vi "Main.vi"(11 "Module Admin":refnum<class "Delacor_lib_QMH_Cloneable Module Admin.lvclass">) -> ()   [LabVIEW 2025, in "Sequencer.lvlib"]
doc: "This template is based off of the Queued Message Handler design pattern and the Queued Message Handler project template that ships with LabVIEW.\n\nThe main difference is that the queue is private to this module and communication between modules is performed via Broadcast and Request events.\n\nRequest events are wrapped in public API methods and are handled in the Event Handling Loop (EHL) of this VI. Any module can register for Broadcast events sent by this module. The EHL generates messages based on user interface actions.\n\nThe Message Handling Loop (MHL) processes messages generated by the EHL, or by other messages. The messages are string values, so new messages can be added easily to the Message Cases case structure in the MHL. Each message cluster can also provide an optional value for Message Data, which is a variant that can be converted to whatever message-specific data is required.\n_____\nBased on DQMH Dev Tools: Project Template 7.1.2.1547."
uses:
  Sequencer.lvlib
  <vilib>/Delacor/Delacor QMH/Libraries/Cloneable Module Admin_class/Delacor_lib_QMH_Cloneable Module Admin.lvclass
  C:/Program Files/National Instruments/LabVIEW 2025/vi.lib/Delacor/Delacor QMH/Libraries/Module Admin_class/Delacor_lib_QMH_Module Admin.lvclass
  Module Data--cluster.ctl
  <vilib>/Delacor/Delacor QMH/Libraries/Message Queue_class/Delacor_lib_QMH_Message Queue.lvclass/Delacor_lib_QMH_Message Queue.ctl
  <vilib>/Delacor/Delacor QMH/Libraries/Cloneable Module Admin_class/Delacor_lib_QMH_Cloneable Module Admin.lvclass/Delacor_lib_QMH_Cloneable Module Admin.ctl
  Stop Argument--cluster.ctl
  <vilib>/Delacor/Delacor QMH/Libraries/Module Admin_class/Delacor_lib_QMH_Module Admin.lvclass/Delacor_lib_QMH_Module Admin.ctl
  Get Modules Argument--cluster.ctl
  Get Modules (Reply Payload)--cluster.ctl
  Home Stepper Argument--cluster.ctl
  Home Stepper (Reply Payload)--cluster.ctl
  Go To Angle Argument--cluster.ctl
  Controls/Angle Indicator.ctl
  Controls/Motor Speed Slider.ctl
  Go To Angle (Reply Payload)--cluster.ctl
  Part Removal Position Argument--cluster.ctl
  Part Removal Position (Reply Payload)--cluster.ctl
  Torque Test Argument--cluster.ctl
  Controls/Sequencer/sequence array.ctl
  Controls/Sequencer/step cluster.ctl
  Torque Test (Reply Payload)--cluster.ctl
  Controls/Sequencer/results array.ctl
  Controls/Sequencer/results cluster.ctl
  <vilib>/Utility/miscctls.llb/LVPointTypeDef.ctl
  <vilib>/Delacor/Delacor QMH/Libraries/Message Queue_class/Delacor_lib_QMH_Enqueue Message (Single).vi
  <vilib>/Delacor/Delacor QMH/Libraries/Cloneable Module Admin_class/Delacor_lib_QMH_Get Module ID.vi
  <vilib>/Delacor/Delacor QMH/Libraries/Module Admin_class/Delacor_lib_QMH_Get External Launch.vi
  <vilib>/Analysis/baseanly.llb/Mean (DBL).vi
  <vilib>/Delacor/Delacor QMH/Libraries/Message Queue_class/Delacor_lib_QMH_Message Queue.lvclass
  USB IO/USB IO.lvlib
  Motor/Motor.lvlib
  <vilib>/Analysis/NI_AALBase.lvlib
  Wheatstone Bridge/Wheatstone Bridge.lvlib
panel:
  out "error out":errorcluster
  out "Status":string
  in  "Simulate EHL Error":bool
  in  "Simulate MHL Error":bool
  # "Other processes communicate with this Module via its Public API (wrappers for its Request Events).\n\nThis Module communicates with other processes via its Broadcast Events.\nAny process that wants to receive these messages can register for this module's Broadcast events."
  # "This template is for the DQMH framework. See the block diagram for more information on how to use this template."
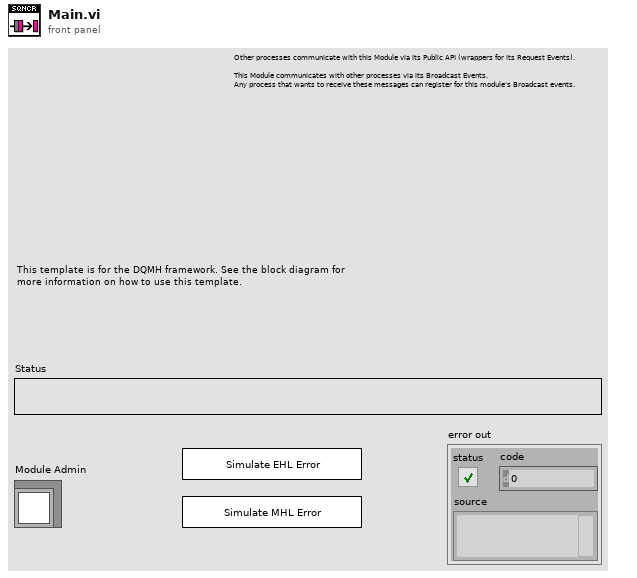
[diagram p1: front panel]
types:
  T1 = typedef "Sequencer.lvlib/Request Events--cluster.ctl" = cluster{"Stop Module":refnum<user-event>, "Show Panel":refnum<user-event>, "Hide Panel":refnum<user-event>, "Show Diagram":refnum<user-event>, "Get Module Execution Status":refnum<user-event>, "Get Modules":refnum<user-event>, "Home":refnum<user-event>, "Home Stepper":refnum<user-event>, "Go To Angle":refnum<user-event>, "Part Removal Position":refnum<user-event>, "Torque Test":refnum<user-event>}
  T2 = typedef "Sequencer.lvlib/Module Data--cluster.ctl" = cluster{"Status":string, "Modules":cluster{"Module IDs":i32[], "Module Names":string[]}}
  T3 = enum32{"invalid lock state", "Not Locked", "Locked (No Password)", "Password-protected"}
  T4 = typedef "Sequencer.lvlib/Stop Argument--cluster.ctl" = cluster{"Module ID":i32, "Origin":string, "Exit via Stop Module Req?":bool, "Wait for Module to stop?":bool}
  T5 = typedef "Sequencer.lvlib/Get Modules Argument--cluster.ctl" = cluster{"Module ID":i32, "Modules":cluster{"Module IDs":i32[], "Module Names":string[]}, "Wait Notifier":refnum<notifier>, "wait for reply":bool}
  T6 = typedef "Sequencer.lvlib/Home Stepper Argument--cluster.ctl" = cluster{"Module ID":i32, "Wait Notifier":refnum<notifier>, "wait for reply":bool}
  T7 = typedef "Sequencer.lvlib/Go To Angle Argument--cluster.ctl" = cluster{"Module ID":i32, "Angle":T8, "Speed [rpm]":T9, "Wait Notifier":refnum<notifier>, "wait for reply":bool}
  T8 = typedef "Angle Indicator.ctl" = dbl
  T9 = typedef "Motor Speed Slider.ctl" = dbl
  T10 = typedef "Sequencer.lvlib/Part Removal Position Argument--cluster.ctl" = cluster{"Module ID":i32, "Wait Notifier":refnum<notifier>, "wait for reply":bool}
  T11 = typedef "Sequencer.lvlib/Torque Test Argument--cluster.ctl" = cluster{"Module ID":i32, "Array 2":T12, "Speed [rpm]":T9, "On Time [ms]":dbl, "Wait Notifier":refnum<notifier>, "wait for reply":bool}
  T12 = typedef "sequence array.ctl" = T13[]
  T13 = typedef "step cluster.ctl" = cluster{"Angle Min [°]":dbl, "Angle Max [°]":dbl, "Torque Min [oz-in]":dbl, "Torque Max [oz-in]":dbl}
  T14 = typedef "LVPointTypeDef.ctl" = cluster{"Horizontal":i16, "Vertical":i16}
  T15 = enum32{"Invalid", "Standard", "Closed", "Hidden", "Minimized", "Maximized"}
  T16 = typedef "Sequencer.lvlib/Get Modules (Reply Payload)--cluster.ctl" = cluster{"Module ID":i32, "error":errorcluster}
  T17 = typedef "Sequencer.lvlib/Home Stepper (Reply Payload)--cluster.ctl" = cluster{"Module ID":i32, "Complete?":bool, "error":errorcluster}
  T18 = typedef "Sequencer.lvlib/Go To Angle (Reply Payload)--cluster.ctl" = cluster{"Module ID":i32, "Complete?":bool, "error":errorcluster}
  T19 = typedef "Sequencer.lvlib/Part Removal Position (Reply Payload)--cluster.ctl" = cluster{"Module ID":i32, "Completed?":bool, "error":errorcluster}
  T20 = typedef "Sequencer.lvlib/Torque Test (Reply Payload)--cluster.ctl" = cluster{"Module ID":i32, "Array 2":T21, "Complete?":bool, "error":errorcluster}
  T21 = typedef "results array.ctl" = T22[]
  T22 = typedef "results cluster.ctl" = cluster{"Angle [°]":dbl, "Torque [oz-in]":dbl, "Pass?":bool}
  T23 = cluster{"Module IDs":i32[], "Module Names":string[]}
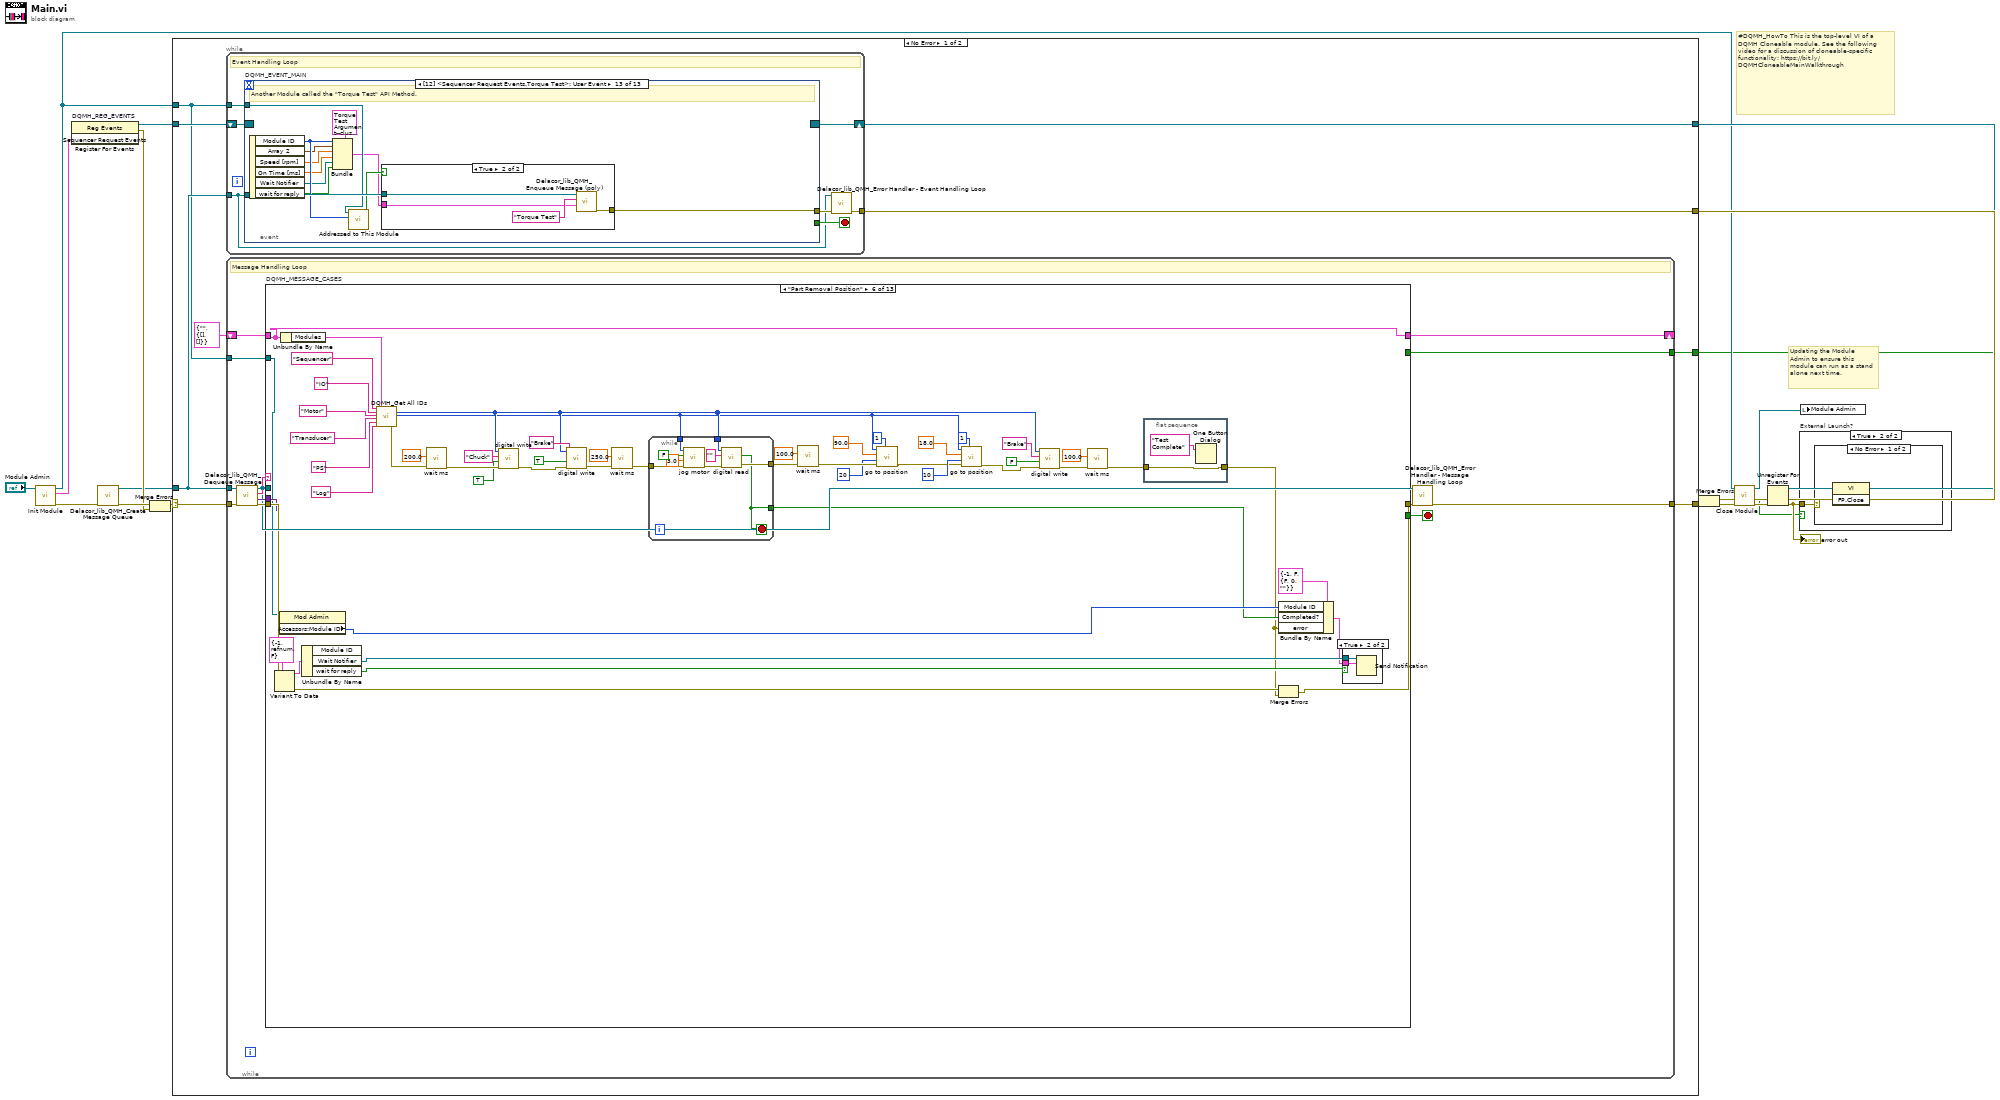
[diagram p0: block diagram]
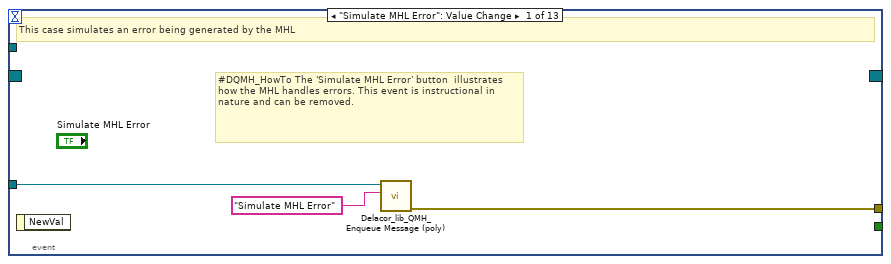
[diagram p2: hidden frame]
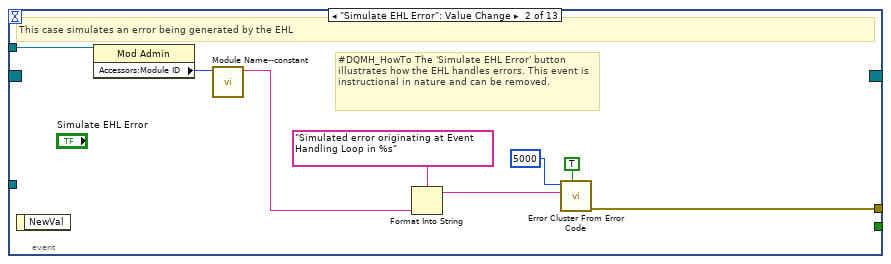
[diagram p3: hidden frame]
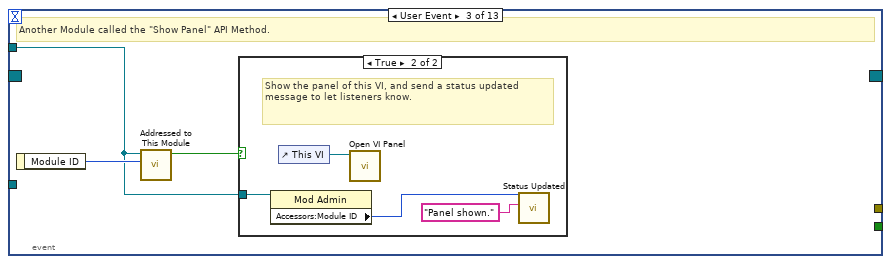
[diagram p4: hidden frame]
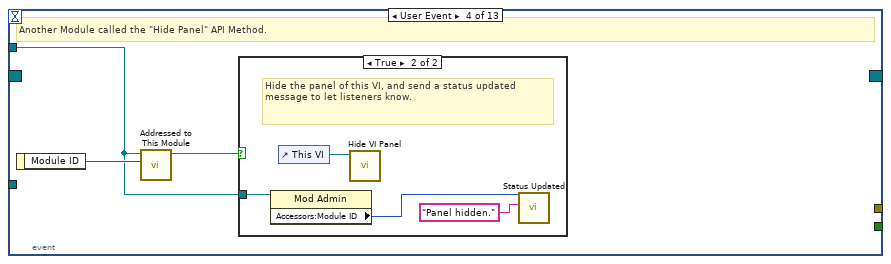
[diagram p6: hidden frame]
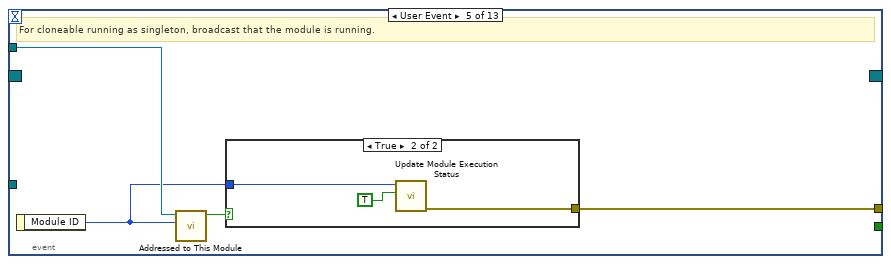
[diagram p8: hidden frame]
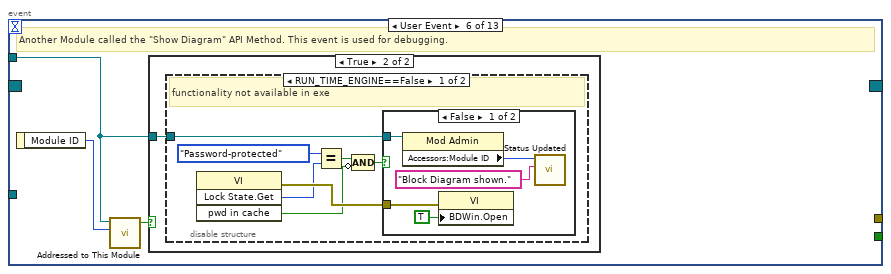
[diagram p10: hidden frame]
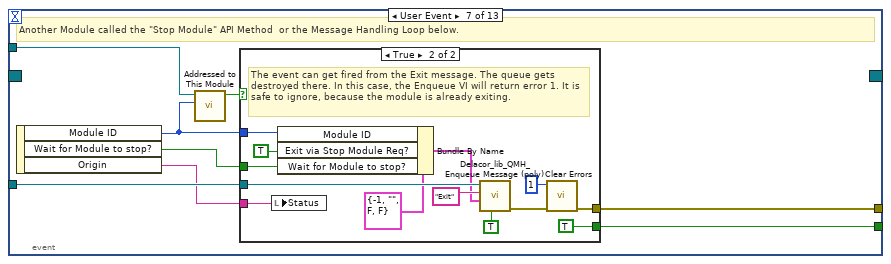
[diagram p14: hidden frame]
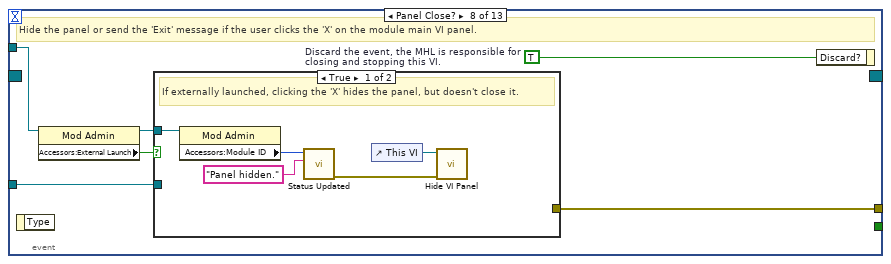
[diagram p16: hidden frame]
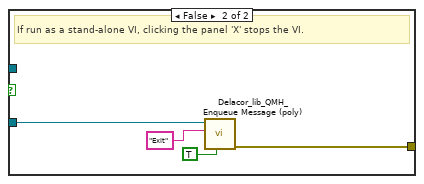
[diagram p17: hidden frame]
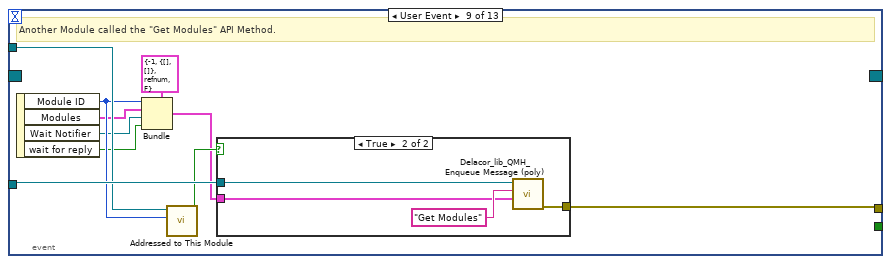
[diagram p18: hidden frame]
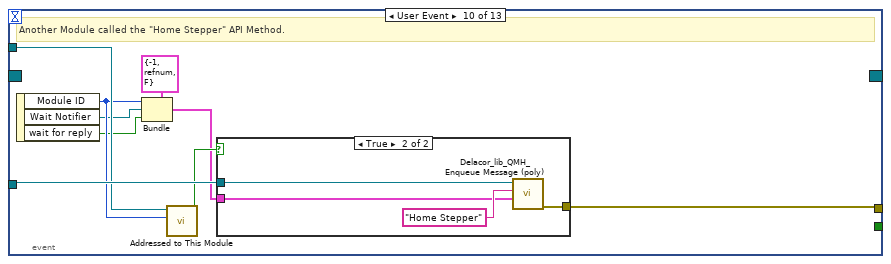
[diagram p20: hidden frame]
diagram:
  # "#DQMH_HowTo This is the top-level VI of a DQMH Cloneable module. See the following video for a discussion of cloneable-specific functionality: https://bit.ly/DQMHCloneableMainWalkthrough"
  # "Updating the Module Admin to ensure this module can run as a stand alone next time."
  n1 = call "Init Module.vi"("Cloneable Module Admin in"="Module Admin") -> ("error out"=w15:errorcluster, "Sequencer Request Events"=w7:T1, "Cloneable Module Admin out"=w4:refnum<class "Delacor_lib_QMH_Cloneable Module Admin.lvclass">)  [unwired: 8 in]
  n2 = register-events "DQMH_REG_EVENTS"(w7) -> (reference out=w8:refnum<event-registration>, error out=w10:errorcluster)  [unwired: 2 in]
  n3 = call <vilib>:"Delacor_lib_QMH_Create Message Queue.vi"("error in"=w15) -> ("error out"=w12:errorcluster, "Message Queue"=w6:refnum<class "Delacor_lib_QMH_Message Queue.lvclass">)  [unwired: 9 in]
  n4 = Merge Errors(w12, w10) -> (w11:errorcluster)
  n5 = case shown="No Error" w11 {
    selector: w11 -> [w25 w595]
    tunnel: [w27 w594] -> w16
    tunnel: [w24 w593] -> w9
    tunnel: w8 -> [w22 w593]
    tunnel: w6 -> [w21 w586]
    tunnel: [w26 _] -> w17
    tunnel: w4 -> [w20 w589]
    tunnel: [w19 _] -> w2
    frame No Error {
      n6 = while {
        tunnel: w21 -> [w28]
        shift-right: [w31] -> w24
        shift-left: w22 -> [w32]
        tunnel: [w33] -> w26
        tunnel: w20 -> [w29]
        stop <- w30 stop-if-true
        # "Event Handling Loop"
        n7 = event "DQMH_EVENT_MAIN" shown="[12] <Sequencer Request Events.Torque Test>: User Event" {
          selector: w32 -> [_ _ _ _ _ _ _ _ _ _ _ _ _]
          dyn-events: [_ _ _ _ _ _ _ _ _ _ _ _ _] -> w31
          timeout: _ -> [_ _ _ _ _ _ _ _ _ _ _ _ _]
          tunnel: [_ _ _ _ _ _ w86 _ _ _ _ _ _] -> w30
          tunnel: w28 -> [w36 _ _ _ _ _ w89 w106 w128 w141 w156 w169 w185]
          tunnel: [w37 w45 _ _ w63 _ w90 w109 w119 w133 w146 w161 w174] -> w34
          tunnel: w29 -> [_ w44 w46 w53 w61 w67 w88 w107 w126 w139 w154 w167 w183]
          event "Simulate MHL Error": Value Change {
            # "#DQMH_HowTo The 'Simulate MHL Error' button  illustrates how the MHL handles errors. This event is instructional in nature and can be removed."
            # "This case simulates an error being generated by the MHL"
            n8 = event-data() -> ()  [unwired: 1 in, 1 out]
            n9 = call-poly <vilib>:"Delacor_lib_QMH_Enqueue Message (poly).vi"("Message"="Simulate MHL Error", "Message Queue in"=w36) -> ("error out"=w37:errorcluster)  [unwired: 8 in, 1 out]
          }
          event "Simulate EHL Error": Value Change {
            # "#DQMH_HowTo The 'Simulate EHL Error' button  illustrates how the EHL handles errors. This event is instructional in nature and can be removed."
            # "This case simulates an error being generated by the EHL"
            n10 = event-data() -> ()  [unwired: 1 in, 1 out]
            n11 = property on="Property Node" class="Mod Admin"(reference=w44) -> ("Accessors:Module ID"=w43:i32)  [unwired: 1 in, 2 out]
            n12 = call "Module Name--constant.vi"("Module ID"=w43) -> ("Module Name"=w38:string)  [unwired: 10 in]
            n13 = Format Into String(format string="Simulated error originating at Event Handling Loop in %s", w38) -> (resulting string=w41:string)  [unwired: 2 in, 1 out]
            n14 = call <vilib>:"Error Cluster From Error Code.vi"("show call chain? (False)"=TRUE, "error message (\"\")"=w41, "error code (0)"=5000) -> ("error out"=w45:errorcluster)  [unwired: 6 in]
          }
          event User Event {
            # "Another Module called the \"Show Panel\" API Method."
            n15 = event-data() -> ("Module ID"=w47:i32)  [unwired: 1 in]
            n16 = call "Addressed to This Module.vi"("Module ID from Argument"=w47, "Module Admin"=w46) -> ("Addressed to this instance?"=w48:bool)  [unwired: 8 in, 1 out]
            n17 = case shown="True" w48 {
              tunnel: w46 -> [_ w50]
              frame False {
              }
              frame True {
                # "Show the panel of this VI, and send a status updated message to let listeners know."
                n18 = property on="Property Node" class="Mod Admin"(reference=w50) -> ("Accessors:Module ID"=w49:i32)  [unwired: 1 in, 2 out]
                n19 = control-ref of="This VI"() -> (w52:refnum<vi>)
                n20 = call "Open VI Panel.vi"("VI"=w52) -> ()  [unwired: 10 in, 1 out]
                n21 = call "Status Updated.vi"("Status"="Panel shown." ("format string"), "Module ID"=w49) -> ()  [unwired: 9 in, 1 out]
              }
            }
          }
          event User Event {
            # "Another Module called the \"Hide Panel\" API Method."
            n22 = event-data() -> ("Module ID"=w54:i32)  [unwired: 1 in]
            n23 = call "Addressed to This Module.vi"("Module ID from Argument"=w54, "Module Admin"=w53) -> ("Addressed to this instance?"=w55:bool)  [unwired: 8 in, 1 out]
            n24 = case shown="True" w55 {
              tunnel: w53 -> [_ w57]
              frame False {
              }
              frame True {
                # "Hide the panel of this VI, and send a status updated message to let listeners know."
                n25 = property on="Property Node" class="Mod Admin"(reference=w57) -> ("Accessors:Module ID"=w56:i32)  [unwired: 1 in, 2 out]
                n26 = control-ref of="This VI"() -> (w59:refnum<vi>)
                n27 = call "Hide VI Panel.vi"("VI"=w59) -> ()  [unwired: 10 in, 1 out]
                n28 = call "Status Updated.vi"("Status"="Panel hidden." ("format string"), "Module ID"=w56) -> ()  [unwired: 9 in, 1 out]
              }
            }
          }
          event User Event {
            # "For cloneable running as singleton, broadcast that the module is running."
            n29 = event-data() -> ("Module ID"=w60:i32)  [unwired: 1 in]
            n30 = call "Addressed to This Module.vi"("Module ID from Argument"=w60, "Module Admin"=w61) -> ("Addressed to this instance?"=w62:bool)  [unwired: 8 in, 1 out]
            n31 = case shown="True" w62 {
              tunnel: [_ w66] -> w63
              tunnel: w60 -> [_ w65]
              frame False {
              }
              frame True {
                n32 = call "Update Module Execution Status.vi"("Running?"=TRUE, "Module ID"=w65) -> ("error out"=w66:errorcluster)  [unwired: 9 in]
              }
            }
          }
          event User Event {
            # "Another Module called the \"Show Diagram\" API Method. This event is used for debugging."
            n33 = event-data() -> ("Module ID"=w68:i32)  [unwired: 1 in]
            n34 = call "Addressed to This Module.vi"("Module ID from Argument"=w68, "Module Admin"=w67) -> ("Addressed to this instance?"=w69:bool)  [unwired: 8 in, 1 out]
            n35 = case shown="True" w69 {
              tunnel: w67 -> [_ w70]
              frame False {
              }
              frame True {
                n36 = disable-structure shown="RUN_TIME_ENGINE==False" {
                  disable-tunnel: w70 -> [w71 _]
                  frame condition #0 (active) {
                    # "functionality not available in exe"
                    n37 = invoke on="Invoke Node" class="VI" method="Lock State.Get"() -> (error out=w77:errorcluster, "Get Lock State"=w76:T3, "pwd in cache"=w73:bool)  [unwired: 4 in, 1 out]
                    n38 = Equal?(x=T3."Password-protected", y=w76) -> (x = y?=w74:bool)
                    n39 = Compound Arithmetic op=AND(w74, invert w73) -> (w72:bool)
                    n40 = case shown="False" w72 {
                      tunnel: w77 -> [w82 _]
                      tunnel: w71 -> [w79 _]
                      frame False {
                        n41 = property on="Property Node" class="Mod Admin"(reference=w79) -> ("Accessors:Module ID"=w78:i32)  [unwired: 1 in, 2 out]
                        n42 = property on="Property Node" class="VI"(error in=w82, "BDWin.Open"=TRUE ("Block Diagram Window:Open")) -> ()  [unwired: 1 in, 2 out]
                        n43 = call "Status Updated.vi"("Status"="Block Diagram shown." ("format string"), "Module ID"=w78) -> ()  [unwired: 9 in, 1 out]
                      }
                      frame True {
                        # "Password-protected VI, and the password is not in the cache. Do not show the diagram."
                      }
                    }
                  }
                  frame condition #1 {
                  }
                }
              }
            }
          }
          event User Event {
            # "Another Module called the \"Stop Module\" API Method  or the Message Handling Loop below."
            n44 = event-data() -> ("Module ID"=w84:i32, "Wait for Module to stop?"=w85:bool, "Origin"=w83:string)  [unwired: 1 in]
            n45 = call "Addressed to This Module.vi"("Module ID from Argument"=w84, "Module Admin"=w88) -> ("Addressed to this instance?"=w87:bool)  [unwired: 8 in, 1 out]
            n46 = case shown="True" w87 {
              tunnel: [_ w102] -> w90
              tunnel: w89 -> [_ w98]
              tunnel: [_ TRUE] -> w86
              tunnel: w85 -> [_ w93]
              tunnel: w84 -> [_ w95]
              tunnel: w83 -> [_ w91]
              frame False {
              }
              frame True {
                # "The event can get fired from the Exit message. The queue gets destroyed there. In this case, the Enqueue VI will return error 1. It is safe to ignore, because the module is already exiting."
                n47 = local write "Status"(w91) -> ()
                n48 = Bundle By Name(cluster=T4 {"Module ID"=-1, "Origin"="", "Exit via Stop Module Req?"=FALSE, "Wait for Module to stop?"=FALSE} ("Stop Argument"), "Module ID"=w95, "Exit via Stop Module Req?"=TRUE, "Wait for Module to stop?"=w93) -> (w92:T4)
                n49 = call-poly <vilib>:"Delacor_lib_QMH_Enqueue Message (poly).vi"("Priority Message? (F)"=TRUE, "Message Data"=w92, "Message"="Exit", "Message Queue in"=w98) -> ("error out"=w103:errorcluster)  [unwired: 6 in, 1 out]
                n50 = call <vilib>:"Clear Errors.vi"("error in (no error)"=w103, "specific error code to clear (0: all)"=1) -> ("error out"=w102:errorcluster)  [unwired: 4 in, 1 out]
              }
            }
          }
          event Panel Close? {
            w108 = TRUE  # Discard the event, the MHL is responsible for closing and stopping this VI.
            # "Hide the panel or send the 'Exit' message if the user clicks the 'X' on the module main VI panel."
            n51 = event-data() -> ()  [unwired: 1 in, 1 out]
            n52 = property on="Property Node" class="Mod Admin"(reference=w107) -> (reference out=w104:refnum<class "Delacor_lib_QMH_Cloneable Module Admin.lvclass">, "Accessors:External Launch"=w105:bool)  [unwired: 1 in, 1 out]
            n53 = case shown="True" w105 {
              tunnel: w106 -> [_ w117]
              tunnel: [_ w118] -> w109
              tunnel: w104 -> [w112 _]
              frame True {
                # "If externally launched, clicking the 'X' hides the panel, but doesn't close it."
                n54 = property on="Property Node" class="Mod Admin"(reference=w112) -> ("Accessors:Module ID"=w111:i32)  [unwired: 1 in, 2 out]
                n55 = call "Status Updated.vi"("Status"="Panel hidden." ("format string"), "Module ID"=w111) -> ("error out"=w110:errorcluster)  [unwired: 9 in]
                n56 = control-ref of="This VI"() -> (w114:refnum<vi>)
                n57 = call "Hide VI Panel.vi"("error in"=w110, "VI"=w114) -> ()  [unwired: 9 in, 1 out]
              }
              frame False {
                # "If run as a stand-alone VI, clicking the panel 'X' stops the VI."
                n58 = call-poly <vilib>:"Delacor_lib_QMH_Enqueue Message (poly).vi"("Priority Message? (F)"=TRUE, "Message"="Exit", "Message Queue in"=w117) -> ("error out"=w118:errorcluster)  [unwired: 7 in, 1 out]
              }
            }
            n59 = event-data ("Event Filter Node")("Discard?"=w108) -> ()  [unwired: 1 in, 1 out]
          }
          event User Event {
            # "Another Module called the \"Get Modules\" API Method."
            n60 = event-data() -> ("Module ID"=w123:i32, "Modules"=w122:T23, "Wait Notifier"=w121:refnum<notifier>, "wait for reply"=w120:bool)  [unwired: 1 in]
            n61 = Bundle(cluster=T5 {"Module ID"=-1, "Modules"={"Module IDs"=[], "Module Names"=[]}, "Wait Notifier"=refnum, "wait for reply"=FALSE} ("Get Modules Argument"), "Module ID"=w123, "Modules"=w122, "Wait Notifier"=w121, "wait for reply"=w120) -> (w124:T5)
            n62 = call "Addressed to This Module.vi"("Module ID from Argument"=w123, "Module Admin"=w126) -> ("Addressed to this instance?"=w127:bool)  [unwired: 8 in, 1 out]
            n63 = case shown="True" w127 {
              tunnel: w128 -> [_ w132]
              tunnel: w124 -> [_ w130]
              tunnel: [_ w129] -> w119
              frame False {
              }
              frame True {
                n64 = call-poly <vilib>:"Delacor_lib_QMH_Enqueue Message (poly).vi"("Message Data"=w130, "Message"="Get Modules", "Message Queue in"=w132) -> ("error out"=w129:errorcluster)  [unwired: 7 in, 1 out]
              }
            }
          }
          event User Event {
            # "Another Module called the \"Home Stepper\" API Method."
            n65 = event-data() -> ("Module ID"=w136:i32, "Wait Notifier"=w135:refnum<notifier>, "wait for reply"=w134:bool)  [unwired: 1 in]
            n66 = Bundle(cluster=T6 {"Module ID"=-1, "Wait Notifier"=refnum, "wait for reply"=FALSE} ("Home Stepper Argument"), "Module ID"=w136, "Wait Notifier"=w135, "wait for reply"=w134) -> (w137:T6)
            n67 = call "Addressed to This Module.vi"("Module ID from Argument"=w136, "Module Admin"=w139) -> ("Addressed to this instance?"=w140:bool)  [unwired: 8 in, 1 out]
            n68 = case shown="True" w140 {
              tunnel: w141 -> [_ w145]
              tunnel: w137 -> [_ w143]
              tunnel: [_ w142] -> w133
              frame False {
              }
              frame True {
                n69 = call-poly <vilib>:"Delacor_lib_QMH_Enqueue Message (poly).vi"("Message Data"=w143, "Message"="Home Stepper", "Message Queue in"=w145) -> ("error out"=w142:errorcluster)  [unwired: 7 in, 1 out]
              }
            }
          }
          event User Event {
            # "Another Module called the \"Go To Angle\" API Method."
            n70 = event-data() -> ("Module ID"=w151:i32, "Angle"=w150:T8, "Speed [rpm]"=w149:T9, "Wait Notifier"=w148:refnum<notifier>, "wait for reply"=w147:bool)  [unwired: 1 in]
            n71 = Bundle(cluster=T7 {"Module ID"=-1, "Angle"=0.0, "Speed [rpm]"=9.818181818181818, "Wait Notifier"=refnum, "wait for reply"=FALSE} ("Go To Angle Argument"), "Module ID"=w151, "Angle"=w150, "Speed [rpm]"=w149, "Wait Notifier"=w148, "wait for reply"=w147) -> (w152:T7)
            n72 = call "Addressed to This Module.vi"("Module ID from Argument"=w151, "Module Admin"=w154) -> ("Addressed to this instance?"=w155:bool)  [unwired: 8 in, 1 out]
            n73 = case shown="True" w155 {
              tunnel: w156 -> [_ w160]
              tunnel: w152 -> [_ w158]
              tunnel: [_ w157] -> w146
              frame False {
              }
              frame True {
                n74 = call-poly <vilib>:"Delacor_lib_QMH_Enqueue Message (poly).vi"("Message Data"=w158, "Message"="Go To Angle", "Message Queue in"=w160) -> ("error out"=w157:errorcluster)  [unwired: 7 in, 1 out]
              }
            }
          }
          event User Event {
            # "Another Module called the \"Part Removal Position\" API Method."
            n75 = event-data() -> ("Module ID"=w164:i32, "Wait Notifier"=w163:refnum<notifier>, "wait for reply"=w162:bool)  [unwired: 1 in]
            n76 = Bundle(cluster=T10 {"Module ID"=-1, "Wait Notifier"=refnum, "wait for reply"=FALSE} ("Part Removal Position Argument"), "Module ID"=w164, "Wait Notifier"=w163, "wait for reply"=w162) -> (w165:T10)
            n77 = call "Addressed to This Module.vi"("Module ID from Argument"=w164, "Module Admin"=w167) -> ("Addressed to this instance?"=w168:bool)  [unwired: 8 in, 1 out]
            n78 = case shown="True" w168 {
              tunnel: w169 -> [_ w173]
              tunnel: w165 -> [_ w171]
              tunnel: [_ w170] -> w161
              frame False {
              }
              frame True {
                n79 = call-poly <vilib>:"Delacor_lib_QMH_Enqueue Message (poly).vi"("Message Data"=w171, "Message"="Part Removal Position", "Message Queue in"=w173) -> ("error out"=w170:errorcluster)  [unwired: 7 in, 1 out]
              }
            }
          }
          event User Event {
            # "Another Module called the \"Torque Test\" API Method."
            n80 = event-data() -> ("Module ID"=w180:i32, "Array 2"=w179:T12, "Speed [rpm]"=w178:T9, "On Time [ms]"=w177:dbl, "Wait Notifier"=w176:refnum<notifier>, "wait for reply"=w175:bool)  [unwired: 1 in]
            n81 = Bundle(cluster=T11 {"Module ID"=-1, "Array 2"=[], "Speed [rpm]"=9.818181818181818, "On Time [ms]"=0.0, "Wait Notifier"=refnum, "wait for reply"=FALSE} ("Torque Test Argument"), "Module ID"=w180, "Array 2"=w179, "Speed [rpm]"=w178, "On Time [ms]"=w177, "Wait Notifier"=w176, "wait for reply"=w175) -> (w181:T11)
            n82 = call "Addressed to This Module.vi"("Module ID from Argument"=w180, "Module Admin"=w183) -> ("Addressed to this instance?"=w184:bool)  [unwired: 8 in, 1 out]
            n83 = case shown="True" w184 {
              tunnel: w185 -> [_ w189]
              tunnel: w181 -> [_ w187]
              tunnel: [_ w186] -> w174
              frame False {
              }
              frame True {
                n84 = call-poly <vilib>:"Delacor_lib_QMH_Enqueue Message (poly).vi"("Message Data"=w187, "Message"="Torque Test", "Message Queue in"=w189) -> ("error out"=w186:errorcluster)  [unwired: 7 in, 1 out]
              }
            }
          }
        }
        n85 = call-dynamic "Delacor_lib_QMH_Error Handler - Event Handling Loop.vi"("error in"=w34, "Message Queue in"=w28) -> ("dup error in"=w33:errorcluster)  [unwired: 8 in, 1 out]
      }
      n86 = while {
        tunnel: w21 -> [w190]
        shift-right: [w197] -> _
        shift-left: T2 {"Status"="", "Modules"={"Module IDs"=[], "Module Names"=[]}} ("Data Cluster") -> [w198]
        tunnel: w25 -> [w201]
        tunnel: [w199] -> w27
        tunnel: w20 -> [w192]
        tunnel: [w191] -> w19
        stop <- w196 stop-if-true
        # "Message Handling Loop"
        n87 = call-dynamic "Delacor_lib_QMH_Dequeue Message.vi"("error in"=w201, "Message Queue in"=w190) -> ("error out"=w200:errorcluster, "Message Data"=w194:variant, "Message"=w195:string, "Message Queue out"=w193:refnum<class "Delacor_lib_QMH_Message Queue.lvclass">)  [unwired: 6 in]
        n88 = case "DQMH_MESSAGE_CASES" shown="\"Part Removal Position\"" w195 {
          selector: w195 -> [_ _ _ _ _ _ _ _ _ _ _ _ w575]
          tunnel: w193 -> [_ _ _ _ _ _ _ _ _ w530 _ w567 _]
          tunnel: w200 -> [w221 w225 w241 w299 w328 w410 w464 w525 w527 w539 w556 w573 w584]
          tunnel: [w219 w225 w232 w290 w319 w401 w455 w524 w527 w535 w555 w568 w585] -> w202
          tunnel: w198 -> [w212 w224 w229 w261 w316 w391 w434 w523 w526 w534 w553 w566 w582]
          tunnel: [w211 w224 w228 w261 w311 w391 w434 w523 w526 w534 w553 w566 w582] -> w197
          tunnel: [_ _ _ _ _ _ _ _ _ _ _ w565 _] -> w196
          tunnel: w194 -> [_ _ w239 w297 w326 w408 w462 _ _ w533 _ w563 _]
          tunnel: w192 -> [w207 _ w230 w288 w317 w399 w453 _ _ w532 w551 w558 w581]
          tunnel: [_ _ _ _ _ _ _ _ _ _ _ w561 _] -> w191
          frame "Initialize" {
            w204 = "Initial Message" ("Initial Message")
            # "#DQMH_CodeNeeded - Initialize the appearance of the front panel."
            # "#DQMH_CodeNeeded - Initialize your state data here."
            # "Initialize - Any operation that needs to be done before the module can receive messages. Synchronize Caller Events.vi will inform Start Module.vi that the module has launched and is ready to receive messages. Module Did Init.vi will broadcast that the module initialized."
            n89 = call "Synchronize Caller Events.vi"("error in"=w221, "Module Admin"=w207) -> ("error out"=w220:errorcluster, "Module Admin out"=w206:refnum<class "Delacor_lib_QMH_Cloneable Module Admin.lvclass">)  [unwired: 8 in]
            n90 = property on="Property Node" class="Mod Admin"(reference=w206) -> ("Accessors:Module ID"=w203:i32, "Accessors:External Launch"=w208:bool)  [unwired: 1 in, 2 out]
            n91 = call "Module Name--constant.vi"("Module ID"=w203) -> ("Module Name"=w216:string)  [unwired: 10 in]
            n92 = property on="Property Node" class="VI"("Front Panel.Title"=w216) -> (reference out=w218:refnum<vi>, error out=w223:errorcluster)  [unwired: 2 in]
            n93 = Select(t=T15."Hidden" ("State"), s=w208, f=T15."Standard" ("State")) -> (s? t:f=w213:T15)
            n94 = invoke on="Invoke Node" class="VI" method="FP.Open"(reference=w218, error in=w223, "State"=w213) -> (reference out=w217:refnum<vi>, error out=w222:errorcluster)  [unwired: 2 in, 3 out]
            n95 = Bundle By Name(cluster=w212, "Status"=w204) -> (w211:T2)
            n96 = invoke on="Invoke Node" class="VI" method="FP.Center"(reference=w217, error in=w222) -> ()  [unwired: 1 in, 3 out]
            n97 = property on="Pane" class="Pane"("Origin"=T14 {"Horizontal"=0, "Vertical"=0}) -> ()  [unwired: 2 in, 2 out]
            n98 = call "Module Name--constant.vi"("Module ID"=w203) -> ("Module Name"=w209:string)  [unwired: 10 in]
            n99 = call "Module Did Init.vi"("error in"=w220, "Initialized?"=TRUE, "Origin"=w209, "Module ID"=w203) -> ("error out"=w219:errorcluster)  [unwired: 7 in]
            "Status" <- w204
          }
          frame "---Module Specific---" {
            # "Separator -- The following cases handle messages specific to this Module."
          }
          frame "Get Modules" {
            n100 = property class="Mod Admin"(reference=w230) -> ("Accessors:Module ID"=w231:i32)  [unwired: 1 in, 2 out]
            n101 = Variant To Data(error in=w241, type=T5 {"Module ID"=-1, "Modules"={"Module IDs"=[], "Module Names"=[]}, "Wait Notifier"=refnum, "wait for reply"=FALSE} ("Get Modules Argument"), Variant=w239) -> (data=w237:T5, error out=w240:errorcluster)
            n102 = Unbundle By Name(w237) -> ("Modules"=w227:T23, "Wait Notifier"=w236:refnum<notifier>, "wait for reply"=w235:bool)  [unwired: 1 out]
            n103 = in-place {
              in-place-border: w227 -> [w243]
              in-place-border: [errorcluster {"status"=FALSE, "code"=0, "source"=""} ("error")] -> w226
              n104 = in-place-cluster #1(w229) -> ()  [unwired: 1 out]
              n105 = in-place-cluster #1("Modules"=w243) -> (w228:T2)
            }
            n106 = Bundle By Name(cluster=T16 {"Module ID"=-1, "error"={"status"=FALSE, "code"=0, "source"=""}} ("Get Modules (Reply Payload)"), "Module ID"=w231, "error"=w226) -> (w234:T16)
            n107 = Merge Errors(w240, w226) -> (w232:errorcluster)
            n108 = case "DQMH_FIRE_NOTIFIER" shown="True" w235 {
              tunnel: w236 -> [_ w245]
              tunnel: w234 -> [_ w244]
              frame False {
              }
              frame True {
                n109 = Send Notification(notification=w244, notifier=w245) -> ()  [unwired: 1 in, 2 out]
              }
            }
          }
          frame "Home Stepper" {
            w251 = 10 ("Pause Time [ms]")
            n110 = property class="Mod Admin"(reference=w288) -> ("Accessors:Module ID"=w289:i32)  [unwired: 1 in, 2 out]
            n111 = Variant To Data(error in=w299, type=T6 {"Module ID"=-1, "Wait Notifier"=refnum, "wait for reply"=FALSE} ("Home Stepper Argument"), Variant=w297) -> (data=w295:T6, error out=w298:errorcluster)
            n112 = Unbundle By Name(w261) -> ("Modules"=w287:T23)
            n113 = Unbundle By Name(w295) -> ("Wait Notifier"=w294:refnum<notifier>, "wait for reply"=w293:bool)  [unwired: 1 out]
            n114 = call "DQMH_Get All IDs.vi"("Module 1"="Sequencer" ("Module Name"), "Module 2"="IO" ("Module Name"), "Module 3"="Motor" ("Module Name"), "Module 4"="Transducer" ("Module Name"), "Module 5"="PS" ("Module Name"), "Module 6"="Log" ("Module Name"), "Modules"=w287) -> ("error out"=w280:errorcluster, "Module 2"=w260:i32, "Module 3"=w246:i32)  [unwired: 6 in, 4 out]
            n115 = call "wait ms.vi"("error in"=w280, "ms (1000)"=200.0) -> ("error out"=w274:errorcluster)  [unwired: 9 in]
            n116 = call "digital write.vi"("error in"=w274, "On/Off"=TRUE, "Line"="Chuck", "Module ID"=w260) -> ("error out"=w273:errorcluster)  [unwired: 6 in, 1 out]
            n117 = call "digital write.vi"("error in"=w273, "On/Off"=TRUE, "Line"="Brake", "Module ID"=w260) -> ("error out"=w276:errorcluster)  [unwired: 6 in, 1 out]
            n118 = call "wait ms.vi"("error in"=w276, "ms (1000)"=250.0) -> ("error out"=w275:errorcluster)  [unwired: 9 in]
            n119 = while {
              tunnel: w275 -> [w308]
              tunnel: w246 -> [w305]
              tunnel: w260 -> [w303]
              tunnel: [w301] -> w248
              tunnel: [w300] -> w249
              stop <- w300 stop-if-true
              n120 = call "jog motor.vi"("error in"=w308, "Speed [rpm]"=2.0, "CCW? (T)"=FALSE, "Module ID"=w305) -> ("error out"=w304:errorcluster)  [unwired: 5 in, 2 out]
              n121 = call "digital read.vi"("error in"=w304, "Line"="", "Module ID"=w303) -> ("error out"=w301:errorcluster, "High/Low"=w300:bool)  [unwired: 6 in, 1 out]
            }
            n122 = call "zero.vi"("error in"=w248, "Module ID"=w246) -> ("error out"=w247:errorcluster)  [unwired: 8 in, 1 out]
            n123 = call "go to position.vi"("Pause Time [ms]"=w251, "error in"=w247, "Velocity [rpm]"=10, "Position"=100.0, "Module ID"=w246) -> ("error out"=w254:errorcluster)  [unwired: 4 in, 2 out]
            n124 = call "go to position.vi"("Pause Time [ms]"=w251, "error in"=w254, "Velocity [rpm]"=5, "Position"=10.0, "Module ID"=w246) -> ("error out"=w250:errorcluster)  [unwired: 4 in, 2 out]
            n125 = call "wait ms.vi"("error in"=w250, "ms (1000)"=100.0) -> ("error out"=w267:errorcluster)  [unwired: 9 in]
            n126 = call "digital write.vi"("error in"=w267, "On/Off"=FALSE, "Line"="Chuck", "Module ID"=w260) -> ("error out"=w265:errorcluster)  [unwired: 6 in, 1 out]
            n127 = call "digital write.vi"("error in"=w265, "On/Off"=FALSE, "Line"="Brake", "Module ID"=w260) -> ("error out"=w262:errorcluster)  [unwired: 6 in, 1 out]
            n128 = call "wait ms.vi"("error in"=w262, "ms (1000)"=100.0) -> ("error out"=w259:errorcluster)  [unwired: 9 in]
            n129 = call "zero.vi"("error in"=w259, "Module ID"=w246) -> ("error out"=w258:errorcluster)  [unwired: 8 in, 1 out]
            n130 = Bundle By Name(cluster=T17 {"Module ID"=-1, "Complete?"=FALSE, "error"={"status"=FALSE, "code"=0, "source"=""}} ("Home Stepper (Reply Payload)"), "Module ID"=w289, "Complete?"=w249, "error"=w258) -> (w292:T17)
            n131 = Merge Errors(w298, w258) -> (w290:errorcluster)
            n132 = case "DQMH_FIRE_NOTIFIER" shown="True" w293 {
              tunnel: w294 -> [_ w310]
              tunnel: w292 -> [_ w309]
              frame False {
              }
              frame True {
                n133 = Send Notification(notification=w309, notifier=w310) -> ()  [unwired: 1 in, 2 out]
              }
            }
          }
          frame "Go To Angle" {
            n134 = Variant To Data(error in=w328, type=T7 {"Module ID"=-1, "Angle"=0.0, "Speed [rpm]"=9.818181818181818, "Wait Notifier"=refnum, "wait for reply"=FALSE} ("Go To Angle Argument"), Variant=w326) -> (data=w324:T7, error out=w327:errorcluster)
            n135 = property class="Mod Admin"(reference=w317) -> ("Accessors:Module ID"=w318:i32)  [unwired: 1 in, 2 out]
            n136 = Unbundle By Name(w324) -> ("Angle"=w315:T8, "Speed [rpm]"=w314:T9, "Wait Notifier"=w323:refnum<notifier>, "wait for reply"=w322:bool)  [unwired: 1 out]
            n137 = in-place {
              in-place-border: w315 -> [w340]
              in-place-border: w314 -> [w339]
              in-place-border: [w331] -> w312
              n138 = in-place-cluster #2(w316) -> ("Modules"=w330:T23)
              n139 = call "DQMH_Get All IDs.vi"("Module 1"="Sequencer" ("Module Name"), "Module 2"="IO" ("Module Name"), "Module 3"="Motor" ("Module Name"), "Module 4"="Transducer" ("Module Name"), "Module 5"="PS" ("Module Name"), "Module 6"="Log" ("Module Name"), "Modules"=w330) -> ("error out"=w351:errorcluster, "Module 2"=w334:i32, "Module 3"=w341:i32)  [unwired: 6 in, 4 out]
              n140 = call "wait ms.vi"("error in"=w351, "ms (1000)"=250.0) -> ("error out"=w350:errorcluster)  [unwired: 9 in]
              n141 = call "digital write.vi"("error in"=w350, "On/Off"=TRUE, "Line"="Brake", "Module ID"=w334) -> ("error out"=w347:errorcluster)  [unwired: 6 in, 1 out]
              n142 = call "digital write.vi"("error in"=w347, "On/Off"=FALSE, "Line"="Chuck", "Module ID"=w334) -> ("error out"=w344:errorcluster)  [unwired: 6 in, 1 out]
              n143 = call "wait ms.vi"("error in"=w344, "ms (1000)"=250.0) -> ("error out"=w342:errorcluster)  [unwired: 9 in]
              n144 = call "go to position.vi"("Pause Time [ms]"=10, "error in"=w342, "Velocity [rpm]"=w339, "Position"=w340, "Module ID"=w341) -> ("error out"=w337:errorcluster)  [unwired: 4 in, 2 out]
              n145 = call "digital write.vi"("error in"=w337, "On/Off"=FALSE, "Line"="Brake", "Module ID"=w334) -> ("error out"=w333:errorcluster)  [unwired: 6 in, 1 out]
              n146 = call "wait ms.vi"("error in"=w333, "ms (1000)"=50.0) -> ("error out"=w331:errorcluster)  [unwired: 9 in]
              n147 = in-place-cluster #2("Modules"=w330) -> (w311:T2)
            }
            n148 = Not(x=w312) -> (.not. x?=w313:bool)
            n149 = Bundle By Name(cluster=T18 {"Module ID"=-1, "Complete?"=FALSE, "error"={"status"=FALSE, "code"=0, "source"=""}} ("Go To Angle (Reply Payload)"), "Module ID"=w318, "Complete?"=w313, "error"=w312) -> (w321:T18)
            n150 = Merge Errors(w327, w312) -> (w319:errorcluster)
            n151 = case "DQMH_FIRE_NOTIFIER" shown="True" w322 {
              tunnel: w323 -> [_ w359]
              tunnel: w321 -> [_ w358]
              frame False {
              }
              frame True {
                n152 = Send Notification(notification=w358, notifier=w359) -> ()  [unwired: 1 in, 2 out]
              }
            }
          }
          frame "Part Removal Position" {
            n153 = Variant To Data(error in=w410, type=T10 {"Module ID"=-1, "Wait Notifier"=refnum, "wait for reply"=FALSE} ("Part Removal Position Argument"), Variant=w408) -> (data=w406:T10, error out=w409:errorcluster)
            n154 = property class="Mod Admin"(reference=w399) -> ("Accessors:Module ID"=w400:i32)  [unwired: 1 in, 2 out]
            n155 = Unbundle By Name(w391) -> ("Modules"=w392:T23)
            n156 = Unbundle By Name(w406) -> ("Wait Notifier"=w405:refnum<notifier>, "wait for reply"=w404:bool)  [unwired: 1 out]
            n157 = call "DQMH_Get All IDs.vi"("Module 1"="Sequencer" ("Module Name"), "Module 2"="IO" ("Module Name"), "Module 3"="Motor" ("Module Name"), "Module 4"="Transducer" ("Module Name"), "Module 5"="PS" ("Module Name"), "Module 6"="Log" ("Module Name"), "Modules"=w392) -> ("error out"=w373:errorcluster, "Module 2"=w374:i32, "Module 3"=w362:i32)  [unwired: 6 in, 4 out]
            n158 = call "wait ms.vi"("error in"=w373, "ms (1000)"=200.0) -> ("error out"=w385:errorcluster)  [unwired: 9 in]
            n159 = call "digital write.vi"("error in"=w385, "On/Off"=TRUE, "Line"="Chuck", "Module ID"=w374) -> ("error out"=w384:errorcluster)  [unwired: 6 in, 1 out]
            n160 = call "digital write.vi"("error in"=w384, "On/Off"=TRUE, "Line"="Brake", "Module ID"=w374) -> ("error out"=w387:errorcluster)  [unwired: 6 in, 1 out]
            n161 = call "wait ms.vi"("error in"=w387, "ms (1000)"=250.0) -> ("error out"=w386:errorcluster)  [unwired: 9 in]
            n162 = while {
              tunnel: w386 -> [w421]
              tunnel: w362 -> [w418]
              tunnel: w374 -> [w416]
              tunnel: [w414] -> w381
              tunnel: [w413] -> w372
              stop <- w413 stop-if-true
              n163 = call "jog motor.vi"("error in"=w421, "Speed [rpm]"=3.0, "CCW? (T)"=FALSE, "Module ID"=w418) -> ("error out"=w417:errorcluster)  [unwired: 5 in, 2 out]
              n164 = call "digital read.vi"("error in"=w417, "Line"="", "Module ID"=w416) -> ("error out"=w414:errorcluster, "High/Low"=w413:bool)  [unwired: 6 in, 1 out]
            }
            n165 = call "wait ms.vi"("error in"=w381, "ms (1000)"=100.0) -> ("error out"=w371:errorcluster)  [unwired: 9 in]
            n166 = call "go to position.vi"("Pause Time [ms]"=1, "error in"=w371, "Velocity [rpm]"=20, "Position"=90.0, "Module ID"=w362) -> ("error out"=w365:errorcluster)  [unwired: 4 in, 2 out]
            n167 = call "go to position.vi"("Pause Time [ms]"=1, "error in"=w365, "Velocity [rpm]"=10, "Position"=18.0, "Module ID"=w362) -> ("error out"=w364:errorcluster)  [unwired: 4 in, 2 out]
            n168 = call "digital write.vi"("error in"=w364, "On/Off"=FALSE, "Line"="Brake", "Module ID"=w374) -> ("error out"=w376:errorcluster)  [unwired: 6 in, 1 out]
            n169 = call "wait ms.vi"("error in"=w376, "ms (1000)"=100.0) -> ("error out"=w361:errorcluster)  [unwired: 9 in]
            n170 = flat-sequence {
              tunnel: w361 -> [w411]
              tunnel: [w411] -> w360
              frame #0 {
                n171 = One Button Dialog(message="Test Complete") -> ()  [unwired: 1 in, 1 out]
              }
            }
            n172 = Bundle By Name(cluster=T19 {"Module ID"=-1, "Completed?"=FALSE, "error"={"status"=FALSE, "code"=0, "source"=""}} ("Part Removal Position (Reply Payload)"), "Module ID"=w400, "Completed?"=w372, "error"=w360) -> (w403:T19)
            n173 = Merge Errors(w409, w360) -> (w401:errorcluster)
            n174 = case "DQMH_FIRE_NOTIFIER" shown="True" w404 {
              tunnel: w405 -> [_ w423]
              tunnel: w403 -> [_ w422]
              frame False {
              }
              frame True {
                n175 = Send Notification(notification=w422, notifier=w423) -> ()  [unwired: 1 in, 2 out]
              }
            }
          }
          frame "Torque Test" {
            n176 = Variant To Data(error in=w464, type=T11 {"Module ID"=-1, "Array 2"=[], "Speed [rpm]"=9.818181818181818, "On Time [ms]"=0.0, "Wait Notifier"=refnum, "wait for reply"=FALSE} ("Torque Test Argument"), Variant=w462) -> (data=w460:T11, error out=w463:errorcluster)
            n177 = property class="Mod Admin"(reference=w453) -> ("Accessors:Module ID"=w454:i32)  [unwired: 1 in, 2 out]
            n178 = Unbundle By Name(w434) -> ("Modules"=w444:T23)
            n179 = Unbundle By Name(w460) -> ("Array 2"=w435:T12, "Speed [rpm]"=w432:T9, "On Time [ms]"=w430:dbl, "Wait Notifier"=w459:refnum<notifier>, "wait for reply"=w458:bool)  [unwired: 1 out]
            n180 = call "DQMH_Get All IDs.vi"("Module 1"="Sequencer" ("Module Name"), "Module 2"="IO" ("Module Name"), "Module 3"="Motor" ("Module Name"), "Module 4"="Transducer" ("Module Name"), "Module 5"="PS" ("Module Name"), "Module 6"="Log" ("Module Name"), "Modules"=w444) -> ("error out"=w445:errorcluster, "Module 2"=w431:i32, "Module 3"=w433:i32, "Module 4"=w424:i32)  [unwired: 6 in, 3 out]
            n181 = call "wait ms.vi"("error in"=w445, "ms (1000)"=200.0) -> ("error out"=w439:errorcluster)  [unwired: 9 in]
            n182 = call "digital write.vi"("error in"=w439, "On/Off"=TRUE, "Line"="Brake", "Module ID"=w431) -> ("error out"=w438:errorcluster)  [unwired: 6 in, 1 out]
            n183 = call "digital write.vi"("error in"=w438, "On/Off"=FALSE, "Line"="Chuck", "Module ID"=w431) -> ("error out"=w436:errorcluster)  [unwired: 6 in, 1 out]
            n184 = call "wait ms.vi"("error in"=w436, "ms (1000)"=250.0) -> ("error out"=w426:errorcluster)  [unwired: 9 in]
            n185 = disable-structure shown="Disabled" {
              disable-tunnel: w426 -> [w467 w468]
              disable-tunnel: [w466 w468] -> w425
              disable-tunnel: w424 -> [w465 _]
              frame Disabled {
                n186 = call "zero.vi"("error in"=w467, "Module ID"=w465) -> ("error out"=w466:errorcluster)  [unwired: 8 in, 1 out]
              }
              frame Enabled {
              }
            }
            n187 = for {
              tunnel: w435 -> [w505] mode=indexing
              tunnel: w433 -> [w488]
              tunnel: w432 -> [w499]
              tunnel: w431 -> [w484]
              tunnel: w424 -> [w492]
              tunnel: [w490] -> w429 mode=indexing
              tunnel: w430 -> [w470]
              shift-right: [w481] -> w428
              shift-left: w425 -> [w501]
              # "For Each Angle"
              n188 = Unbundle By Name(w505) -> ("Angle Min [°]"=w504:dbl, "Angle Max [°]"=w503:dbl, "Torque Min [oz-in]"=w478:dbl, "Torque Max [oz-in]"=w480:dbl)
              n189 = Build Array(w504, w503) -> (w502:dbl[])
              n190 = call-poly <vilib>:"Mean.vi"("X"=w502) -> ("mean"=w500:dbl)  [unwired: 1 out]
              n191 = call "go to position.vi"("Pause Time [ms]"=50, "error in"=w501, "Velocity [rpm]"=w499, "Position"=w500, "Module ID"=w488) -> ("error out"=w497:errorcluster)  [unwired: 4 in, 2 out]
              n192 = call "wait ms.vi"("error in"=w497, "ms (1000)"=20.0) -> ("error out"=w489:errorcluster)  [unwired: 9 in]
              n193 = call "read position.vi"("error in"=w489, "Module ID"=w488) -> ("error out"=w471:errorcluster, "Position"=w487:dbl)  [unwired: 7 in, 1 out]
              n194 = flat-sequence {
                tunnel: w471 -> [_]
                tunnel: w470 -> [w508]
                tunnel: [w509] -> w469
                frame #0 {
                  n195 = Get Date/Time In Seconds() -> (seconds since 1Jan1904=w510:timestamp)
                  n196 = Divide(x=w508, y=1000.0) -> (x/y=w506:dbl)
                  n197 = Add(x=w510, y=w506) -> (x+y=w509:timestamp)
                }
              }
              n198 = Initialize Array(0.0 ("element"), 1 ("dimension size")) -> (w475:dbl[])
              n199 = call "digital write.vi"("error in"=w471, "On/Off"=TRUE, "Line"="PS", "Module ID"=w484) -> ("error out"=w493:errorcluster)  [unwired: 6 in, 1 out]
              n200 = while {
                tunnel: w492 -> [w520]
                shift-right: [w518] -> w474
                shift-left: w475 -> [w519]
                tunnel: w471 -> [w515]
                tunnel: [w514] -> w472
                tunnel: w469 -> [w513]
                i -> [w517]
                stop <- w511 continue-if-true
                # "Torque Recording Loop"
                n201 = Get Date/Time In Seconds() -> (seconds since 1Jan1904=w512:timestamp)
                n202 = call "read dvr.vi"("error in"=w515, "Module ID"=w520) -> ("error out"=w514:errorcluster, "Numeric"=w516:dbl)  [unwired: 7 in, 1 out]
                n203 = Greater?(x=w513, y=w512) -> (0:w511:bool)
                n204 = Insert Into Array(array=w519, index=w517, new element=w516) -> (w518:dbl[])
              }
              n205 = call "wait ms.vi"("error in"=w493, "ms (1000)"=w470) -> ()  [unwired: 9 in, 1 out]
              n206 = call "wait ms.vi"("error in"=w472, "ms (1000)"=40.0) -> ("error out"=w485:errorcluster)  [unwired: 9 in]
              n207 = Array Max & Min(array=w474) -> (max value=w473:dbl)  [unwired: 3 out]
              n208 = call "digital write.vi"("error in"=w485, "On/Off"=FALSE, "Line"="PS", "Module ID"=w484) -> ("error out"=w481:errorcluster)  [unwired: 6 in, 1 out]
              n209 = In Range and Coerce(upper limit=w480, x=w473, lower limit=w478) -> (In Range?=w479:bool)  [unwired: 1 out]
              n210 = Bundle By Name(cluster=T22 {"Angle [°]"=0.0, "Torque [oz-in]"=0.0, "Pass?"=FALSE} ("Cluster"), "Angle [°]"=w487, "Torque [oz-in]"=w473, "Pass?"=w479) -> (w490:T22)
            }
            n211 = Bundle By Name(cluster=T20 {"Module ID"=-1, "Array 2"=[], "Complete?"=FALSE, "error"={"status"=FALSE, "code"=0, "source"=""}} ("Torque Test (Reply Payload)"), "Module ID"=w454, "Array 2"=w429, "Complete?"=TRUE, "error"=w428) -> (w457:T20)
            n212 = Merge Errors(w463, w428) -> (w455:errorcluster)
            n213 = case "DQMH_FIRE_NOTIFIER" shown="True" w458 {
              tunnel: w459 -> [_ w522]
              tunnel: w457 -> [_ w521]
              frame False {
              }
              frame True {
                n214 = Send Notification(notification=w521, notifier=w522) -> ()  [unwired: 1 in, 2 out]
              }
            }
          }
          frame "---Copy This Frame---" {
            # "Duplicate this frame when creating new messages.  Change this comment in the duplicated frame to describe this message."
            n215 = Merge Errors(w525) -> (w524:errorcluster)
          }
          frame "---Exit and Error Handling---" {
            # "Separator - the following cases handle errors and exit messages."
          }
          frame "Error" {
            # "#DQMH_CodeRecommended - If the module is running in standalone mode (External Launch = FALSE), this code will pop up an error dialog and call the 'Exit' message if an error occurs. Add more fine-grained error management here."
            # "Error - Check the error message data and respond accordingly. This message is sent by the \"Error Handler\" VIs at the end of each loop in this application."
            n216 = property on="Property Node" class="Mod Admin"(reference=w532) -> ("Accessors:External Launch"=w531:bool, "Accessors:Module ID"=w529:i32)  [unwired: 1 in, 2 out]
            n217 = Variant To Data(error in=w539, type=errorcluster {"status"=FALSE, "code"=0, "source"=""} ("error constant"), Variant=w533) -> (data=w528:errorcluster, error out=w537:errorcluster)
            n218 = local write "error out"(w528) -> ()
            n219 = call "Error Reported.vi"("Error"=w528, "Module ID"=w529) -> ()  [unwired: 9 in, 1 out]
            n220 = case shown="False" w531 {
              tunnel: [w544 _] -> w536
              tunnel: w530 -> [w542 _]
              tunnel: w528 -> [w543 _]
              frame False {
                n221 = disable-structure shown="Default" {
                  disable-tunnel: w543 -> [w545 _]
                  frame condition #0 (active) {
                    # "If the module is running standalone, then pop up an error dialog and call the \"Exit\" message."
                    n222 = call <vilib>:"Simple Error Handler.vi"("error in (no error)"=w545) -> ()  [unwired: 4 in, 5 out]
                  }
                  frame condition #1 {
                    # "To prevent the Simple Error Handler VI from being loaded (e.g. when deploying to a Real-Time target), add the Conditional Disable Symbol \"DQMH_Disable_SEH\" to your project and set it to TRUE."
                  }
                }
                n223 = call-poly <vilib>:"Delacor_lib_QMH_Enqueue Message (poly).vi"("Priority Message? (F)"=TRUE, "Message"="Exit", "Message Queue in"=w542) -> ("error out"=w544:errorcluster)  [unwired: 7 in, 1 out]
              }
              frame True {
                # "If the module was launched externally, calling the Error Reported broadcast VI is the only action performed by the \"Error\" message. The module's caller can then process the error appropriately."
              }
            }
            n224 = Merge Errors(w537, w536) -> (w535:errorcluster)
          }
          frame "Simulate MHL Error" {
            # "#DQMH_HowTo The 'Simulate MHL Error' button  illustrates how the MHL handles errors. This event is instructional in nature and can be removed."
            # "Simulate an error occurring at the MHL"
            n225 = property on="Property Node" class="Mod Admin"(reference=w551) -> ("Accessors:Module ID"=w552:i32)  [unwired: 1 in, 2 out]
            n226 = call "Module Name--constant.vi"("Module ID"=w552) -> ("Module Name"=w547:string)  [unwired: 10 in]
            n227 = Format Into String(format string="Simulated error originating at Message Handling Loop in %s", w547) -> (resulting string=w548:string)  [unwired: 2 in, 1 out]
            n228 = call <vilib>:"Error Cluster From Error Code.vi"("show call chain? (False)"=TRUE, "error message (\"\")"=w548, "error code (0)"=5001) -> ("error out"=w554:errorcluster)  [unwired: 6 in]
            n229 = Merge Errors(w556, w554) -> (w555:errorcluster)
          }
          frame "Exit" {
            w564 = 91  # 91: not all Exit messages will have an argument
            w565 = TRUE  # Stop the VI
            # "Release the message queue reference"
            # "#DQMH_CodeNeeded - Add any required cleanup code here."
            # "Exit - Exit the application."
            n230 = Variant To Data(error in=w573, type=T4 {"Module ID"=-1, "Origin"="", "Exit via Stop Module Req?"=FALSE, "Wait for Module to stop?"=FALSE} ("Stop Argument"), Variant=w563) -> (data=w560:T4, error out=w569:errorcluster)
            n231 = call <vilib>:"Clear Errors.vi"("error in (no error)"=w569, "specific error code to clear (0: all)"=w564) -> ("error out"=w572:errorcluster)  [unwired: 4 in, 1 out]
            n232 = property on="Property Node" class="Mod Admin"(reference=w558) -> ("Accessors:Module ID"=w557:i32)  [unwired: 1 in, 2 out]
            n233 = control-ref of="This VI"() -> (w559:refnum<vi>)
            n234 = call-dynamic "Delacor_lib_QMH_Release Message Queue.vi"("error in"=w572, "Message Queue"=w567) -> ("error out"=w571:errorcluster)  [unwired: 9 in]
            n235 = call "Handle Exit.vi"("Stop Argument"=w560, "Module Admin in"=w558, "VI reference"=w559) -> ("error out"=w570:errorcluster, "Wait for Stop?"=w561:bool)  [unwired: 7 in]
            n236 = Merge Errors(w571, w570) -> (w568:errorcluster)
            n237 = call "Error Reported.vi"("Error"=w568, "Module ID"=w557) -> ()  [unwired: 9 in, 1 out]
          }
          frame Default {
            # "'Default' case only runs if there is a message that isn't defined in any of the other cases.  Output a programming error."
            n238 = property on="Property Node" class="Mod Admin"(reference=w581) -> ("Accessors:Module ID"=w580:i32)  [unwired: 1 in, 2 out]
            n239 = call "Module Name--constant.vi"("Module ID"=w580) -> ("Module Name"=w574:string)  [unwired: 10 in]
            n240 = Format Into String(format string="The invalid message string \"%s\" was received in the Message Handling Loop for module \"%s\".", w575, w574) -> (resulting string=w577:string)  [unwired: 2 in, 1 out]
            n241 = call <vilib>:"Error Cluster From Error Code.vi"("show call chain? (False)"=TRUE, "error message (\"\")"=w577, "error code (0)"=1) -> ("error out"=w583:errorcluster)  [unwired: 6 in]
            n242 = Merge Errors(w584, w583) -> (w585:errorcluster)
          }
        }
        n243 = call-dynamic "Delacor_lib_QMH_Error Handler - Message Handling Loop.vi"("error in"=w202, "Message Queue in"=w193) -> ("dup error in"=w199:errorcluster)  [unwired: 8 in, 1 out]
      }
    }
    frame Error {
      n244 = call "Synchronize Caller Events.vi"("Module Admin"=w589) -> ("Module Admin out"=w588:refnum<class "Delacor_lib_QMH_Cloneable Module Admin.lvclass">)  [unwired: 9 in, 1 out]
      n245 = property on="Property Node" class="Mod Admin"(reference=w588) -> ("Accessors:Module ID"=w587:i32)  [unwired: 1 in, 2 out]
      n246 = call-dynamic "Delacor_lib_QMH_Release Message Queue.vi"("error in"=w595, "Message Queue"=w586) -> ("error out"=w594:errorcluster)  [unwired: 9 in]
      n247 = call "Module Name--constant.vi"("Module ID"=w587) -> ("Module Name"=w592:string)  [unwired: 10 in]
      n248 = Format Into String(format string="An error occurred during initialization. %s is no longer running.", w592) -> (resulting string=w590:string)  [unwired: 2 in, 1 out]
      n249 = call "Error Reported.vi"("Additional Information"=w590, "Error"=w594, "Module ID"=w587) -> ()  [unwired: 8 in, 1 out]
    }
  }
  n250 = Merge Errors(w17, w16) -> (w18:errorcluster)
  n251 = call "Close Module.vi"("error in"=w18, "Wait for stop?"=w2, "Module Admin in"=w4) -> ("error out"=w14:errorcluster, "External Launch"=w1:bool, "Module Admin out"=w3:refnum<class "Delacor_lib_QMH_Cloneable Module Admin.lvclass">)  [unwired: 6 in]
  n252 = Unregister For Events(event registration refnum=w9, error in=w14) -> (error out=w13:errorcluster)
  "error out" <- w13
  n253 = case "External Launch?" shown="True" w1 {
    tunnel: w13 -> [_ w596]
    frame False {
    }
    frame True {
      n254 = case shown="No Error" w596 {
        frame No Error {
          n255 = invoke class="VI" method="FP.Close"() -> ()  [unwired: 3 in, 3 out]
        }
        frame Error {
          n256 = disable-structure shown="Default" {
            frame condition #0 (active) {
              n257 = invoke class="VI" method="FP.Open"("Activate"=TRUE ("Activate?")) -> ()  [unwired: 4 in, 5 out]
            }
            frame condition #1 {
              # "Don't show panel on error if running inside a built EXE."
            }
          }
        }
      }
    }
  }
  n258 = local write "Module Admin"(w3) -> ()
